vi "Get All Panels.vi"(8 "error in (no error)":errorcluster, 11 "Manager in":refnum<class "Manager.lvclass">) -> (0 "error out":errorcluster, 2 "Panels":refnum<class "Panel.lvclass">[](array[class]), 3 "Manager out":refnum<class "Manager.lvclass">)   [LabVIEW 2020, in "OOPanel.lvlib" / "Manager.lvclass"]
uses:
  Manager.lvclass
  Panel/Panel.lvclass
  Manager.lvclass/Manager.ctl
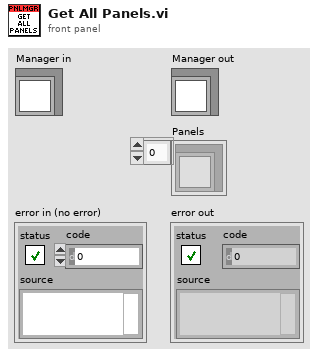
[diagram p1: front panel]
types:
  T1 = typedef "OOPanel.lvlib/Manager.lvclass/Ref Data.ctl" = cluster{"Created Panels":refnum<class "Panel.lvclass">[], "Subpanel Map":map{refnum<vi>, T2}}
  T2 = typedef "OOPanel.lvlib/Manager.lvclass/Subpanel Data.ctl" = cluster{"Panel":refnum<class "Panel.lvclass">, "Has Panel":bool, "Visible":bool}
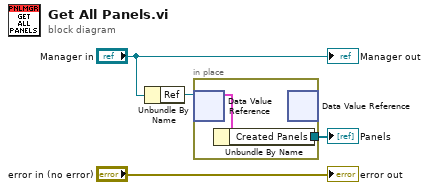
[diagram p0: block diagram]
diagram:
  n1 = Unbundle By Name("Manager in") -> ("Ref"=w3:refnum<data-value>)
  n2 = in-place {
    in-place-border: [w5] -> w1
    n3 = in-place-dvr #1(w3) -> (w6:T1)  [unwired: 1 out]
    n4 = Unbundle By Name(w6) -> ("Created Panels"=w5:refnum<class "Panel.lvclass">[])
    n5 = in-place-dvr #1() -> ()  [unwired: 1 in, 2 out]
  }
  "Panels" <- w1
  "error out" <- "error in (no error)"
  "Manager out" <- "Manager in"
